vi "T_ACC.vi"(1 "最慢周期":i32, 2 "最快周期":i32, 3 "步數":i32) -> (0 "週期":u32[](array[numeric]))   [LabVIEW 2019]
panel:
  out "Waveform Chart 2":i32[](graph)
  in  "加速度":i32
  out "Waveform Chart":u32[](graph)
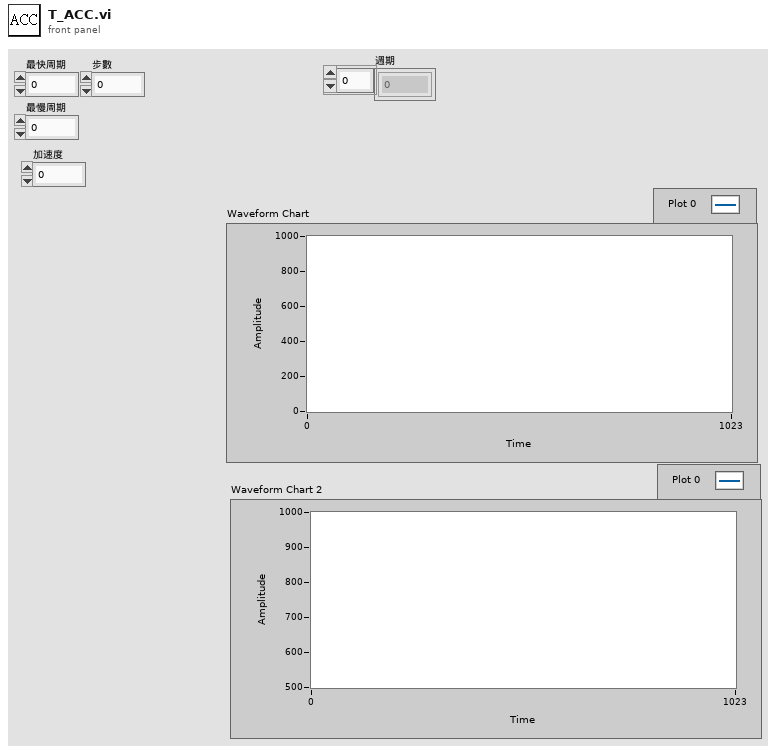
[diagram p1: front panel]
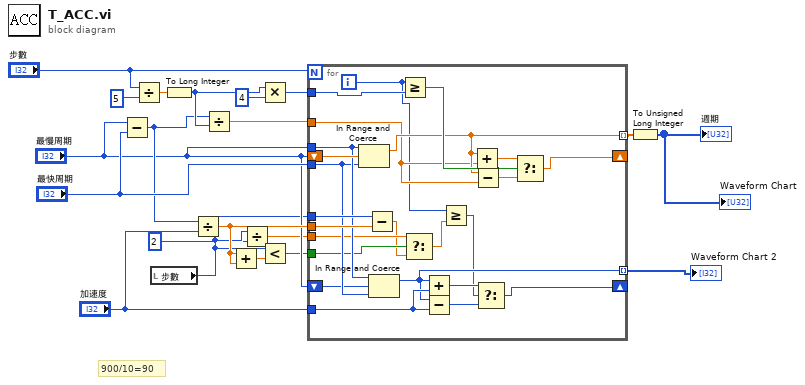
[diagram p0: block diagram]
diagram:
  # "900/10=90"
  n1 = Subtract(x="最慢周期", y="最快周期") -> (x-y=w10:i32)
  n2 = Divide(x="步數", y=5) -> (x/y=w17:dbl)
  n3 = local read "步數"() -> (w3:i32)
  n4 = To Long Integer(number=w17) -> (32bit integer=w15:i32)
  n5 = Divide(x=w10, y="加速度") -> (x/y=w9:dbl)
  n6 = Divide(x=w10, y=w15) -> (x/y=w13:dbl)
  n7 = Add(x=w9, y=w9) -> (x+y=w8:dbl)
  n8 = Divide(x=w3, y=2) -> (x/y=w1:dbl)
  n9 = Multiply(x=w15, y=4) -> (x*y=w16:i32)
  n10 = Less?(x=w3, y=w8) -> (x < y?=w4:bool)
  n11 = for {
    N: "步數" -> [_]
    tunnel: "最快周期" -> [w32]
    tunnel: "最慢周期" -> [w33]
    shift-right: [w38] -> _
    shift-left: "最慢周期" -> [w44]
    tunnel: [w41] -> w12 mode=indexing
    tunnel: w16 -> [w37]
    tunnel: w13 -> [w40]
    tunnel: w9 -> [w34]
    tunnel: w3 -> [w35]
    shift-right: [w27] -> _
    shift-left: "最慢周期" -> [w31]
    tunnel: "加速度" -> [w30]
    tunnel: [w26] -> w5 mode=indexing
    tunnel: w4 -> [w25]
    tunnel: w1 -> [w23]
    i -> [w36]
    n12 = In Range and Coerce(upper limit=w33, x=w44, lower limit=w32) -> (coerced(x)=w41:dbl)  [unwired: 1 out]
    n13 = Subtract(x=w35, y=w34) -> (x-y=w22:dbl)
    n14 = In Range and Coerce(upper limit=w33, x=w31, lower limit=w32) -> (coerced(x)=w26:i32)  [unwired: 1 out]
    n15 = Greater Or Equal?(x=w36, y=w37) -> (x >= y?=w43:bool)
    n16 = Select(t=w23, s=w25, f=w22) -> (s? t:f=w21:dbl)
    n17 = Add(x=w26, y=w30) -> (x+y=w29:i32)
    n18 = Subtract(x=w26, y=w30) -> (x-y=w28:i32)
    n19 = Greater Or Equal?(x=w36, y=w21) -> (x >= y?=w24:bool)
    n20 = Add(x=w41, y=w40) -> (x+y=w42:dbl)
    n21 = Subtract(x=w41, y=w40) -> (x-y=w39:dbl)
    n22 = Select(t=w29, s=w24, f=w28) -> (s? t:f=w27:i32)
    n23 = Select(t=w42, s=w43, f=w39) -> (s? t:f=w38:dbl)
  }
  "Waveform Chart 2" <- w5
  n24 = To Unsigned Long Integer(number=w12) -> (unsigned 32bit integer=→"週期" →"Waveform Chart":u32[])
